vi "py_venv_init.vi"() -> (3 "Refnum out":refnum<k35>)   [LabVIEW 2023]
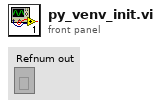
[diagram p1: front panel]
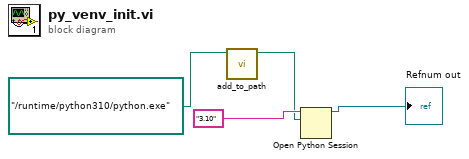
[diagram p0: block diagram]
diagram:
  n1 = call "add_to_path.vi"("Path"=path "../runtime/python310/python.exe") -> ("appended path"=w2:path)  [unwired: 10 in]
  n2 = Open Python Session(python version="3.10", python path=w2) -> (session out=→"Refnum out":refnum<k35>)  [unwired: 1 in, 1 out]
